vi "Refresh from Plots Config.vi"(8 "error in (no error)":errorcluster, 11 "HistorianCharting in":refnum<class "HistorianCharting.lvclass">) -> (0 "error out":errorcluster, 3 "HistorianCharting out":refnum<class "HistorianCharting.lvclass">)   [LabVIEW 2020, in "VolatusGUIElements.lvlib" / "HistorianCharting.lvclass"]
uses:
  HistorianCharting.lvclass
  HistorianCharting.lvclass/HistorianCharting.ctl
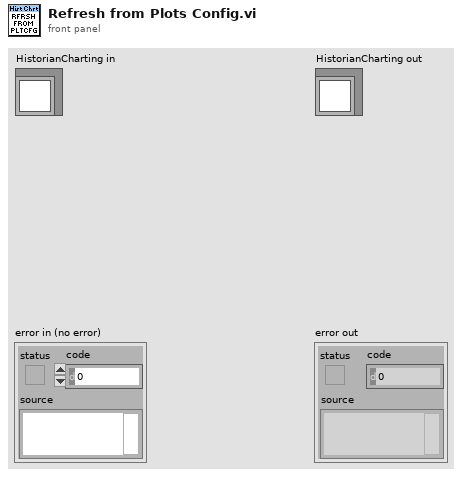
[diagram p1: front panel]
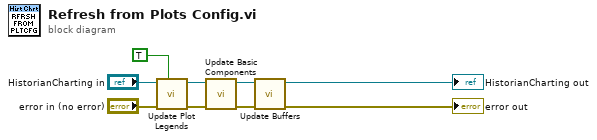
[diagram p0: block diagram]
diagram:
  n1 = call "Update Plot Legends.vi"("Update Config (F)"=TRUE, "error in (no error)"="error in (no error)", "HistorianCharting in"="HistorianCharting in") -> ("error out"=w8:errorcluster, "HistorianCharting out"=w6:refnum<class "HistorianCharting.lvclass">)  [unwired: 7 in]
  n2 = call "Update Basic Components.vi"("error in (no error)"=w8, "HistorianCharting in"=w6) -> ("error out"=w5:errorcluster, "HistorianCharting out"=w3:refnum<class "HistorianCharting.lvclass">)  [unwired: 8 in]
  n3 = call "Update Buffers.vi"("error in (no error)"=w5, "HistorianCharting in"=w3) -> ("error out"=→"error out":errorcluster, "HistorianCharting out"=→"HistorianCharting out":refnum<class "HistorianCharting.lvclass">)  [unwired: 8 in]
